vi "Test Generate Mock Class Replaces Class Control and Constant.vi"(8 "error in (no error)":errorcluster, 11 "Test Case In":refnum<class "_Mock Class Generator Test.lvclass">) -> (0 "error out":errorcluster, 3 "Test Case Out":refnum<class "_Mock Class Generator Test.lvclass">)   [LabVIEW 2020, in "_Mock Class Generator Test.lvclass"]
uses:
  _Mock Class Generator Test.lvclass
  C:/Program Files (x86)/National Instruments/LabVIEW 2020/vi.lib/Astemes/LUnit/Test Case.lvclass
  <vilib>/Astemes/LUnit/Test Case.lvclass/Test Case.ctl
  source/Scripting/Mock Class Generator/Mock Class Generator.lvclass
  <vilib>/Astemes/LUnit/Test Case.lvclass
panel:
  out "No error?":bool
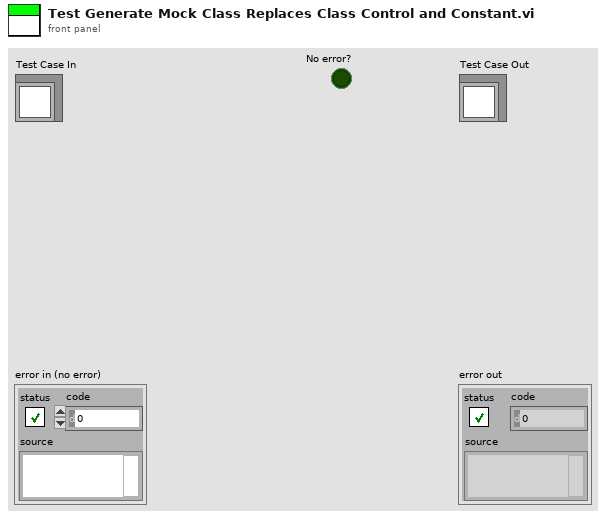
[diagram p1: front panel]
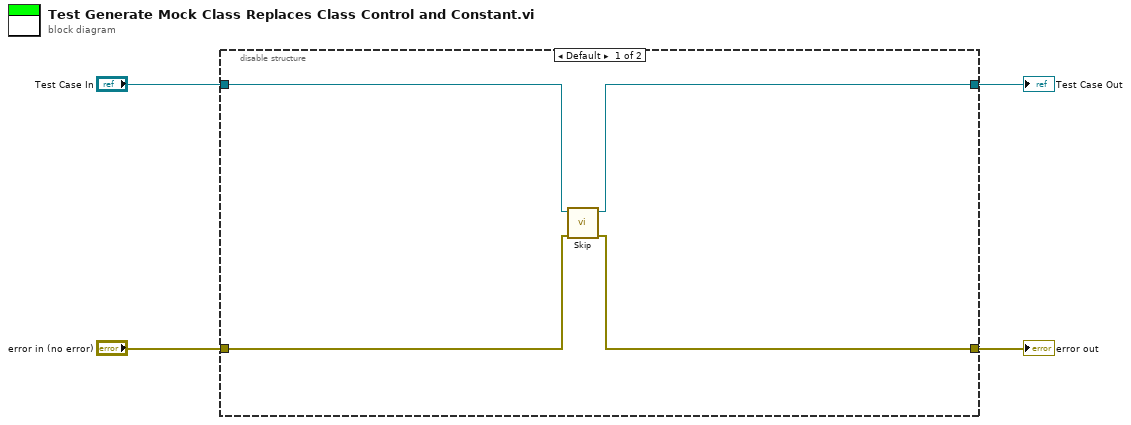
[diagram p0: block diagram]
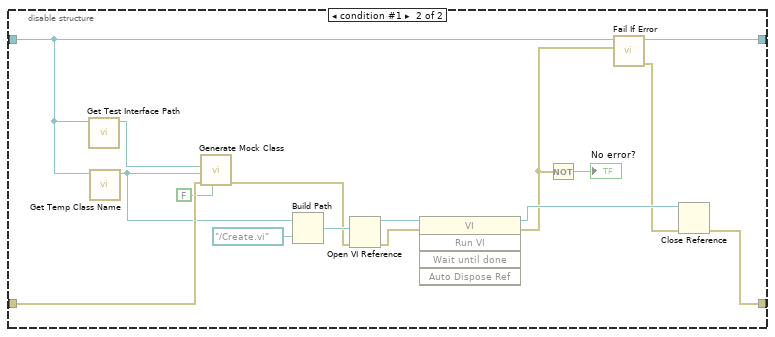
[diagram p2: hidden frame]
diagram:
  n1 = disable-structure shown="Default" {
    disable-tunnel: [w6 w24] -> w4
    disable-tunnel: "Test Case In" -> [w8 w22]
    disable-tunnel: "error in (no error)" -> [w7 w21]
    disable-tunnel: [w5 w11] -> w1
    frame condition #0 (active) {
      n2 = call <vilib>:"Skip.vi"("error in (no error)"=w7, "LUnit Test Case In"=w8) -> ("error out"=w5:errorcluster, "LUnit Test Case Out"=w6:refnum<class "_Mock Class Generator Test.lvclass">)  [unwired: 8 in]
    }
    frame condition #1 {
      n3 = call "Get Test Interface Path.vi"("Mock Class Generator Test in"=w22) -> ("Test Class Path"=w23:path)  [unwired: 10 in]
      n4 = call "Get Temp Class Name.vi"("Mock Class Generator Test in"=w22) -> ("Test Class Path"=w19:path)  [unwired: 10 in]
      n5 = call "Generate Mock Class.vi"("Add to lvproj?"=FALSE, "error in (no error)"=w21, "Destination Class Path"=w19, "Source Class Path"=w23) -> ("error out"=w14:errorcluster)  [unwired: 6 in, 1 out]
      n6 = Build Path(base path=w19, name or relative path=path "../Create.vi") -> (appended path=w17:path)
      n7 = Open VI Reference(vi path=w17, error in (no error)=w14) -> (vi reference=w16:refnum<vi>, error out=w15:errorcluster)  [unwired: 4 in]
      n8 = invoke class="VI" method="Run VI"(reference=w16, error in=w15) -> (reference out=w13:refnum<vi>, error out=w10:errorcluster)  [unwired: 3 in, 3 out]
      n9 = Not(x=w10) -> (.not. x?=→"No error?":bool)
      n10 = call <vilib>:"Fail If Error.vi"("Assert error"=w10, "LUnit Test Case In"=w22) -> ("error out"=w12:errorcluster, "LUnit Test Case Out"=w24:refnum<class "_Mock Class Generator Test.lvclass">)  [unwired: 8 in]
      n11 = Close Reference(reference=w13, error in (no error)=w12) -> (error out=w11:errorcluster)
    }
  }
  "error out" <- w1
  "Test Case Out" <- w4
